vi "KeyboardSerializer.vi"(11 "Sample Number":u32) -> (2 "Keyboard No Op":bool, 3 "SerializedKeyPress":T1)   [LabVIEW 2026, in "dependencies.lvlib"]
uses:
  dependencies.lvlib
  KeyboardLUTSelector.ctl
  <userlib>/_OpenG.lib/boolean/boolean.llb/openg_boolean__ogtk.lvlib
  <userlib>/_OpenG.lib/comparison/comparison.llb/openg_comparison__ogtk.lvlib
  SerializedKeyPress.ctl
  KeyType.ctl
  <userlib>/_OpenG.lib/comparison/comparison.llb/I16 Changed__ogtk.vi
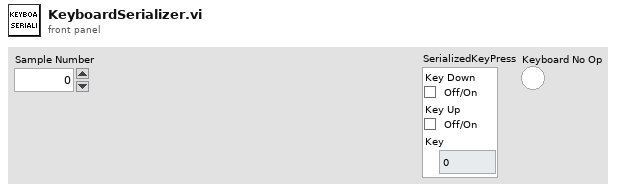
[diagram p1: front panel]
types:
  T1 = typedef "dependencies.lvlib/SerializedKeyPress.ctl" = cluster{"Key Down":bool, "Key Up":bool, "Key":T2}
  T2 = typedef "dependencies.lvlib/KeyType.ctl" = enum16{"0", "1", "2", "3", "4", "5", "6", "7", "8", "9", "A", "B", "C", "D", "E", "F", "G", "H", "I", "J", "K", "L", "M", "N", "O", "P", "Q", "R", "S", "T", "U", "V", "W", "X", "Y", "Z", "F1", "F2", "F3", "F4", "F5", "F6", "F7", "F8", "F9", "F10", "F11", "F12", "F13", "F14", "F15", "ADD", "BACK", "BACKSLASH", "CAPITAL", "COMMA", "DECIMAL", "DELETE", "DIVIDE", "DOWN", "END", "EQUALS", "ESCAPE", "GRAVE (`)", "HOME", "INSERT", "LBRACKET", "LCONTROL", "LEFT", "L ALT", "LSHIFT", "LWIN", "MINUS", "MULTIPLY", "NEXT", "NUMLOCK", "NUMPAD_0", "NUMPAD_1", "NUMPAD_2", "NUMPAD_3", "NUMPAD_4", "NUMPAD_5", "NUMPAD_6", "NUMPAD_7", "NUMPAD_8", "NUMPAD_9", "PAUSE", "PERIOD", "PRIOR (PG UP)", "RBRACKET", "RCONTROL", "RETURN", "RIGHT", "R ALT", "RSHIFT", "RWIN", "SCROLL", "SEMICOLON", "SLASH", "SPACE", "SUBTRACT", "TAB", "UP", "ENTER (num pad)", "' (quote)"}
  T3 = typedef "dependencies.lvlib/KeyboardLUTSelector.ctl" = enum16{"Initialize", "Get Keyboards Keys Pressed at Sample Number", "Assign Keyboard Key Press to Sample Number"}
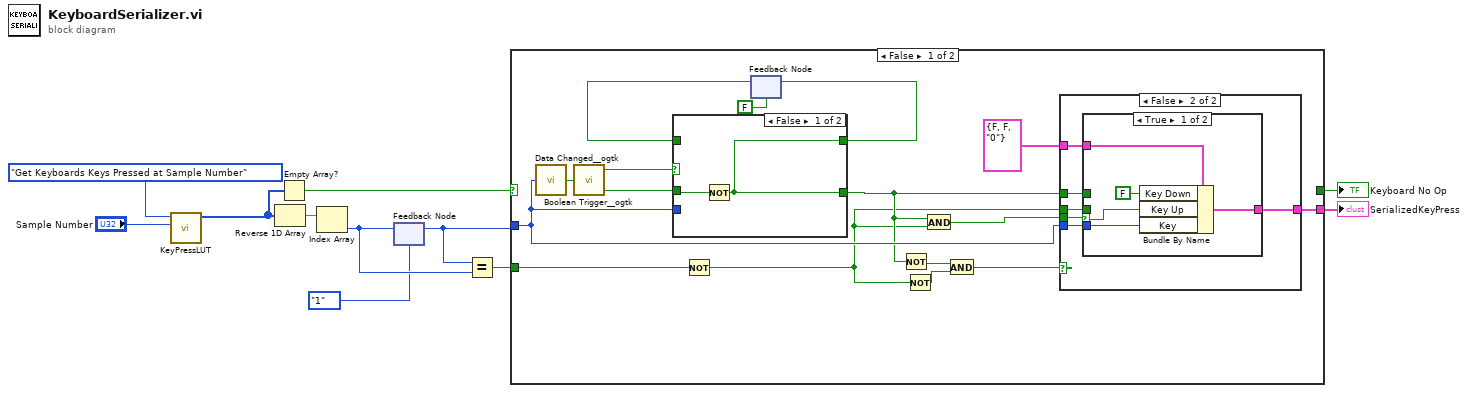
[diagram p0: block diagram]
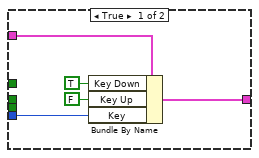
[diagram p2: hidden frame]
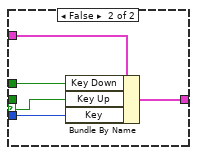
[diagram p3: hidden frame]
diagram:
  n1 = call "KeyPressLUT.vi"("Sample Number"="Sample Number", "LUT Selector"=KeyboardLUTSelector."Get Keyboards Keys Pressed at Sample Number") -> ("KeyboardKeysPressed"=w7:T2[])  [unwired: 8 in, 1 out]
  n2 = Reverse 1D Array(array=w7) -> (reversed array=w10:T2[])
  n3 = Empty Array?(array=w7) -> (empty?=w8:bool)
  n4 = Index Array(array=w10) -> (element=w4:T2)  [unwired: 1 in]
  n5 = feedback #1(KeyType."1" ("keyType Recorded")) -> (w3:T2)
  n6 = feedback-in #1(w4) -> ()
  n7 = Equal?(x=w3, y=w4) -> (x = y?=w9:bool)
  n8 = case shown="False" w8 {
    selector: w8 -> [_ w53]
    tunnel: [w27 _] -> w5
    tunnel: w3 -> [w20 _]
    tunnel: w9 -> [w13 _]
    tunnel: [_ w53] -> w2
    frame False {
      n9 = call-poly <userlib>:"Data Changed__ogtk.vi"("I16"=w20) -> ("Changed"=w26:bool)
      n10 = call <userlib>:"Boolean Trigger__ogtk.vi"("Boolean Input"=w26) -> ("Rising Edge"=w25:bool, "Falling Edge"=w21:bool)  [unwired: 1 in]
      n11 = Not(x=w13) -> (.not. x?=w16:bool)
      n12 = feedback #2(FALSE ("Rising Edge")) -> (w23:bool)
      n13 = case shown="False" w25 {
        selector: w25 -> [_ w52]
        tunnel: w23 -> [_ _]
        tunnel: [w49 w52] -> w22
        tunnel: w20 -> [_ _]
        tunnel: w21 -> [w50 w51]
        tunnel: [w49 w51] -> w18
        frame False {
          n14 = Not(x=w50) -> (.not. x?=w49:bool)
        }
        frame True {
        }
      }
      n15 = feedback-in #2(w22) -> ()
      n16 = Not(x=w18) -> (.not. x?=w17:bool)
      n17 = Not(x=w16) -> (.not. x?=w15:bool)
      n18 = And(x=w18, y=w16) -> (x .and. y?=w19:bool)
      n19 = And(x=w17, y=w15) -> (x .and. y?=w14:bool)
      n20 = case shown="False" w14 {
        tunnel: [w32 w38] -> w27
        tunnel: w20 -> [w31 w37]
        tunnel: w19 -> [_ w36]
        tunnel: w18 -> [_ w35]
        tunnel: w16 -> [_ w34]
        tunnel: T1 {"Key Down"=FALSE, "Key Up"=FALSE, "Key"=enum."0"} -> [w28 w33]
        frame True {
          n21 = Bundle By Name(cluster=w28, "Key Down"=TRUE, "Key Up"=FALSE, "Key"=w31) -> (w32:T1)
        }
        frame False {
          n22 = case shown="True" w36 {
            selector: w36 -> [w40 w46]
            tunnel: [w43 w48] -> w38
            tunnel: w37 -> [w42 w47]
            tunnel: w34 -> [_ _]
            tunnel: w35 -> [_ w45]
            tunnel: w33 -> [w39 w44]
            frame True {
              n23 = Bundle By Name(cluster=w39, "Key Down"=FALSE, "Key Up"=w40, "Key"=w42) -> (w43:T1)
            }
            frame False {
              n24 = Bundle By Name(cluster=w44, "Key Down"=w45, "Key Up"=w46, "Key"=w47) -> (w48:T1)
            }
          }
        }
      }
    }
    frame True {
    }
  }
  "SerializedKeyPress" <- w5
  "Keyboard No Op" <- w2
